vi "DAC Configure.vi"(8 "error in":errorcluster, 11 "DAC Jumo DP in":refnum<class "DAC Jumo DP.lvclass">) -> (0 "error out":errorcluster, 3 "DAC Jumo DP out":refnum<class "DAC Jumo DP.lvclass">)   [LabVIEW 2019, in "DAC.lvlib" / "DAC Jumo DP.lvclass"]
uses:
  DAC Jumo DP.lvclass
  C:/Users/wg/Documents/LV_Projects/test-stand/App/DAC/DAC.lvclass
  DAC.lvclass/DAC.ctl
  DAC Jumo DP.lvclass/DAC Jumo DP.ctl
  <vilib>/DAQmx/create/scale.llb/DAQmx Create Scale (Map Ranges).vi
  <vilib>/DAQmx/create/channels.llb/DAQmx Create Channel (AI-Voltage-Basic).vi
  DAC.lvclass
  <resource>/objmgr/daqmx.rc
  <vilib>/DAQmx/configure/timing.llb/DAQmx Timing (Sample Clock).vi
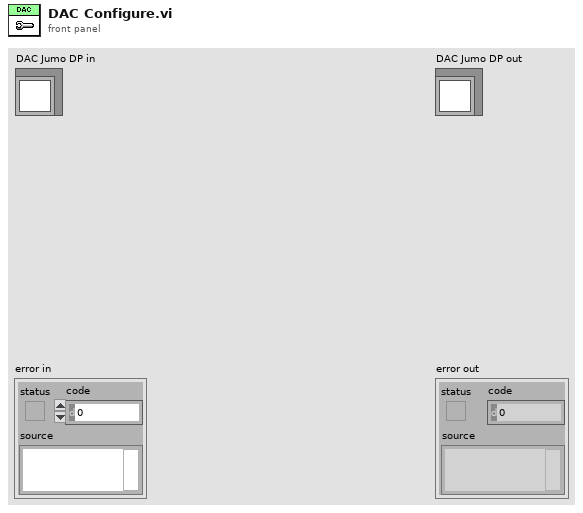
[diagram p1: front panel]
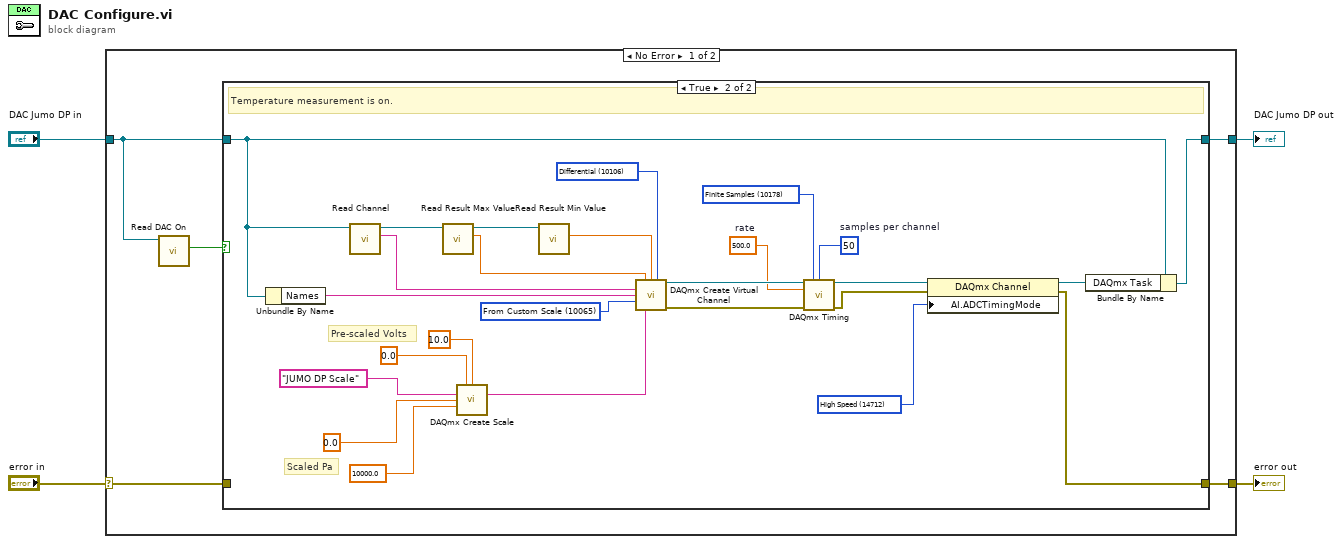
[diagram p0: block diagram]
diagram:
  n1 = case shown="No Error" "error in" {
    selector: "error in" -> [w6 w39]
    tunnel: [w5 w39] -> w4
    tunnel: [w7 w38] -> w3
    tunnel: "DAC Jumo DP in" -> [w9 w38]
    frame No Error {
      n2 = call "Read DAC On.vi"("DAC in"=w9) -> ("DAC On"=w8:bool)  [unwired: 8 in, 2 out]
      n3 = case shown="True" w8 {
        tunnel: w9 -> [w11 w34]
        tunnel: [w11 w37] -> w7
        tunnel: w6 -> [w10 _]
        tunnel: [w10 w13] -> w5
        frame False {
          # "Temperature measurement is off."
        }
        frame True {
          w17 = 500.0  # rate
          w18 = 50  # samples per channel
          w19 = 10178 items=["Finite Samples"=10178, "Continuous Samples"=10123, "Hardware Timed Single Point"=12522] ("sample mode")
          w22 = 10106 items=["Default"=-1, "RSE"=10083, "NRSE"=10078, "Differential"=10106, "Pseudodifferential"=12529] ("input terminal configuration")
          w29 = 10065 items=["Volts"=10348, "From Custom Scale"=10065] ("units")
          w35 = 14712 items=["Automatic"=16097, "High Resolution"=10195, "High Speed"=14712, "Best 50 Hz Rejection"=14713, "Best 60 Hz Rejection"=14714, "Custom"=10137] ("AI.ADCTimingMode")
          # "Scaled Pa"
          # "Pre-scaled Volts"
          # "Temperature measurement is on."
          n4 = Unbundle By Name(w34) -> ("Names"=w36:string)
          n5 = call "Read Channel.vi"("DAC in"=w34) -> ("Channel"=w12:string, "DAC out"=w33:refnum<class "DAC Jumo DP.lvclass">)  [unwired: 8 in, 1 out]
          n6 = call "Read Result Max Value.vi"("DAC in"=w33) -> ("Max Value"=w30:dbl, "DAC out"=w32:refnum<class "DAC Jumo DP.lvclass">)  [unwired: 8 in, 1 out]
          n7 = call-poly <vilib>:"DAQmx Create Scale.vi"("pre-scaled minimum"=0.0, "pre-scaled maximum"=10.0, "name"="JUMO DP Scale", "scaled minimum"=0.0, "scaled maximum"=10000.0) -> ("scale out"=w23:tag)  [unwired: 9 in, 1 out]
          n8 = call "Read Result Min Value.vi"("DAC in"=w32) -> ("Min Value"=w31:dbl)  [unwired: 8 in, 2 out]
          n9 = call-poly <vilib>:"DAQmx Create Virtual Channel.vi"("maximum value"=w30, "minimum value"=w31, "input terminal configuration"=w22, "physical channels"=w12, "name to assign"=w36, "units"=w29, "custom scale name"=w23) -> ("task out"=w21:refnum<k21>, "error out"=w16:errorcluster)  [unwired: 7 in]
          n10 = call-poly <vilib>:"DAQmx Timing.vi"("task/channels in"=w21, "sample mode"=w19, "samples per channel"=w18, "rate"=w17, "error in"=w16) -> ("task out"=w20:refnum<k21>, "error out"=w14:errorcluster)  [unwired: 9 in]
          n11 = property class="DAQmx Channel"(reference=w20, error in=w14, "AI.ADCTimingMode"=w35) -> (reference out=w15:refnum<k21>, error out=w13:errorcluster)
          n12 = Bundle By Name(cluster=w34, "DAQmx Task"=w15) -> (w37:refnum<class "DAC Jumo DP.lvclass">)
        }
      }
    }
    frame Error {
    }
  }
  "error out" <- w4
  "DAC Jumo DP out" <- w3
